vi "Read Paperless Recorder File.vi"(11 "Path":path=path "E:/BaiduSyncdisk/曲线生成/原始曲线/5-1 无纸记录仪 6通道.xls") -> (3 "Data Series":T1[](array[typedef]))   [LabVIEW 2020, in "Data Viewer.lvlib"]
uses:
  Data Viewer.lvlib
  Data Serie--cluster.ctl
  File Type--enum.ctl
  <vilib>/Utility/file.llb/Read Delimited Spreadsheet (string).vi
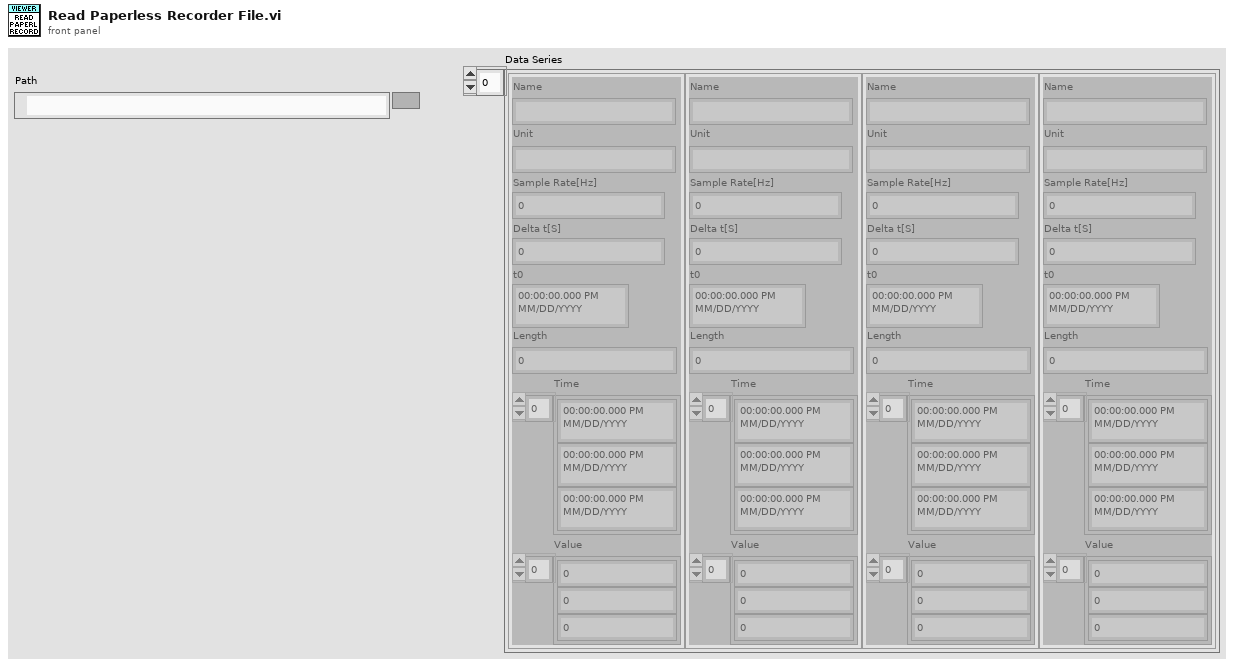
[diagram p1: front panel]
types:
  T1 = typedef "Data Viewer.lvlib/Data Serie--cluster.ctl" = cluster{"Name":string, "Unit":string, "Sample Rate[Hz]":dbl, "Delta t[S]":dbl, "t0":timestamp, "Length":i32, "Time":timestamp[], "Value":dbl[]}
  T2 = typedef "Data Viewer.lvlib/File Type--enum.ctl" = enum16{"伟思环境箱", "增达环境箱", "广五所环境箱", "无纸记录仪", "帕捷SA00339", "记录仪840", "记录仪8400", "记录仪MR888", "*.csv"}
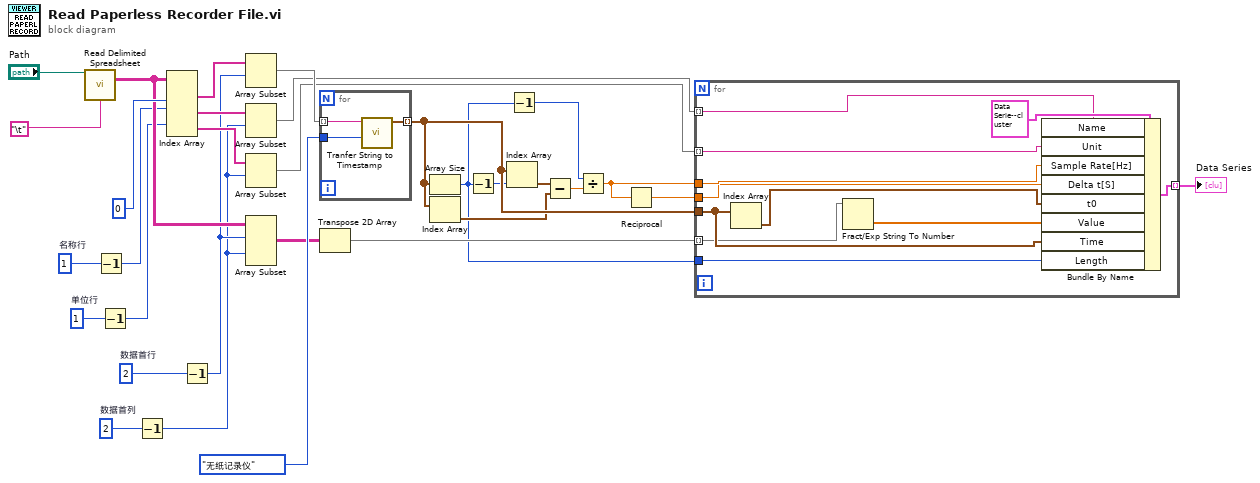
[diagram p0: block diagram]
diagram:
  w22 = 2  # 数据首列
  w23 = 2  # 数据首行
  w25 = 1  # 单位行
  w27 = 1  # 名称行
  n1 = call-poly <vilib>:"Read Delimited Spreadsheet.vi"("file path (dialog if empty)"="Path", "delimiter (\\t)"="\t") -> ("all rows"=w8:string[][])  [unwired: 8 in, 5 out]
  n2 = Decrement(x=w27) -> (x-1=w6:i32)
  n3 = Decrement(x=w25) -> (x-1=w5:i32)
  n4 = Decrement(x=w22) -> (x-1=w3:i32)
  n5 = Index Array(array=w8, index (col) #1=0 ("disabled index (col)"), index (row) #2=w6, index (row) #3=w5) -> (element #1=w30:string[], element #2=w26:string[], element #3=w24:string[])  [unwired: 3 in]
  n6 = Decrement(x=w23) -> (x-1=w4:i32)
  n7 = Array Subset(array=w30, index=w4) -> (w29:string[])  [unwired: 1 in]
  n8 = Array Subset(array=w26, index=w3) -> (w20:string[])  [unwired: 1 in]
  n9 = Array Subset(array=w24, index=w3) -> (w19:string[])  [unwired: 1 in]
  n10 = Array Subset(array=w8, index (row)=w4, index (col)=w3) -> (w21:string[][])  [unwired: 2 in]
  n11 = for {
    tunnel: w29 -> [w34] mode=indexing
    tunnel: File_Type--enum."无纸记录仪" ("File Type") -> [w33]
    tunnel: [w32] -> w17 mode=indexing
    n12 = call "Tranfer String to Timestamp.vi"("File Type"=w33, "String"=w34) -> ("time stamp"=w32:timestamp)  [unwired: 9 in]
  }
  n13 = Transpose 2D Array(2D array=w21) -> (transposed array=w18:string[][])
  n14 = Array Size(array=w17) -> (size(s)=w1:i32)
  n15 = Index Array(array=w17) -> (element=w14:timestamp)  [unwired: 1 in]
  n16 = Decrement(x=w1) -> (x-1=w16:i32)
  n17 = Index Array(array=w17, index=w16) -> (element=w15:timestamp)
  n18 = Decrement(x=w1) -> (x-1=w2:i32)
  n19 = Subtract(x=w15, y=w14) -> (x-y=w13:dbl)
  n20 = Divide(x=w2, y=w13) -> (x/y=w12:dbl)
  n21 = Reciprocal(x=w12) -> (1/x=w11:dbl)
  n22 = for {
    tunnel: w20 -> [w44] mode=indexing
    tunnel: w19 -> [w36] mode=indexing
    tunnel: w18 -> [w41] mode=indexing
    tunnel: w17 -> [w42]
    tunnel: w12 -> [w39]
    tunnel: w11 -> [w38]
    tunnel: [w37] -> w10 mode=indexing
    tunnel: w1 -> [w35]
    n23 = Index Array(array=w42) -> (element=w43:timestamp)  [unwired: 1 in]
    n24 = Fract/Exp String To Number(string=w41) -> (number=w40:dbl[])  [unwired: 3 in, 1 out]
    n25 = Bundle By Name(cluster=T1 {"Name"="", "Unit"="", "Sample Rate[Hz]"=0.0, "Delta t[S]"=0.0, "t0"=timestamp(0 s since 1904-01-01), "Length"=0, "Time"=[], "Value"=[]} ("Data Serie"), "Name"=w44, "Unit"=w36, "Sample Rate[Hz]"=w39, "Delta t[S]"=w38, "t0"=w43, "Value"=w40, "Time"=w42, "Length"=w35) -> (w37:T1)
  }
  "Data Series" <- w10
